vi "wiringPiI2CReadBlockData.vi"(8 "error in (no error)":errorcluster, 9 "values":u8[](array[numeric]), 10 "reg":i32, 11 "devID":T1) -> (0 "error out":errorcluster, 2 "return":i32, 3 "values readed":u8[](array[numeric]))   [LabVIEW 2020, in "wiringPi.lvlib"]
doc: "<b>_______________________________________________________________</b>\n** Author: Juan José Villacorta\n** LabVIEW wrapper for C library <b> wiringPi </b>,\n** https://github.com/WiringPi/WiringPi\n<b>_______________________________________________________________</b>\n\n/*\n * wiringPiI2CReadReg8: wiringPiI2CReadReg16:\n * Read a block of data from a regsiter on the device\n *********************************************************************************\n */"
uses:
  wiringPi.lvlib
  Type Defs/I2C Device.ctl
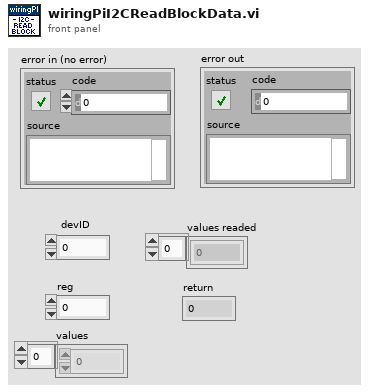
[diagram p1: front panel]
types:
  T1 = typedef "wiringPi.lvlib/I2C Device.ctl" = i32
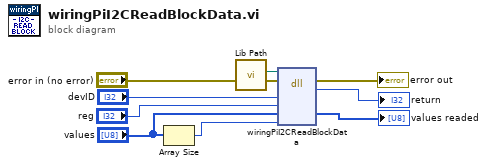
[diagram p0: block diagram]
diagram:
  n1 = Array Size(array="values") -> (size(s)=w2:i32)
  n2 = call "Lib Path.vi"() -> ("path out"=w7:path)  [unwired: 11 in]
  n3 = dll-call lib="libLVwiringPI.so" fn="wiringPiI2CReadBlockData"(path in=w7, error in="error in (no error)", "fd"="devID", "reg"="reg", "values"="values", "size"=w2) -> (error out=→"error out":errorcluster, "return type"=→"return":i32, "values"=→"values readed":u8[])  [unwired: 4 in, 1 out]
